vi "GPIB_SR400_B.vi"(11 "N per point":i32=1) -> (0 "B Gate":dbl[](array[numeric]), 2 "x/y":dbl)   [LabVIEW 2024]
uses:
  <vilib>/Utility/error.llb/Trim Whitespace One-Sided.vi
  GPIB_Address.vi
panel:
  in  "VISA resource name":refnum<visa-resource-name>="GPIB0::23::INSTR"
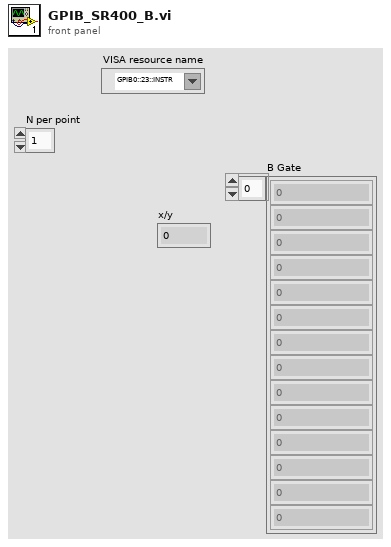
[diagram p1: front panel]
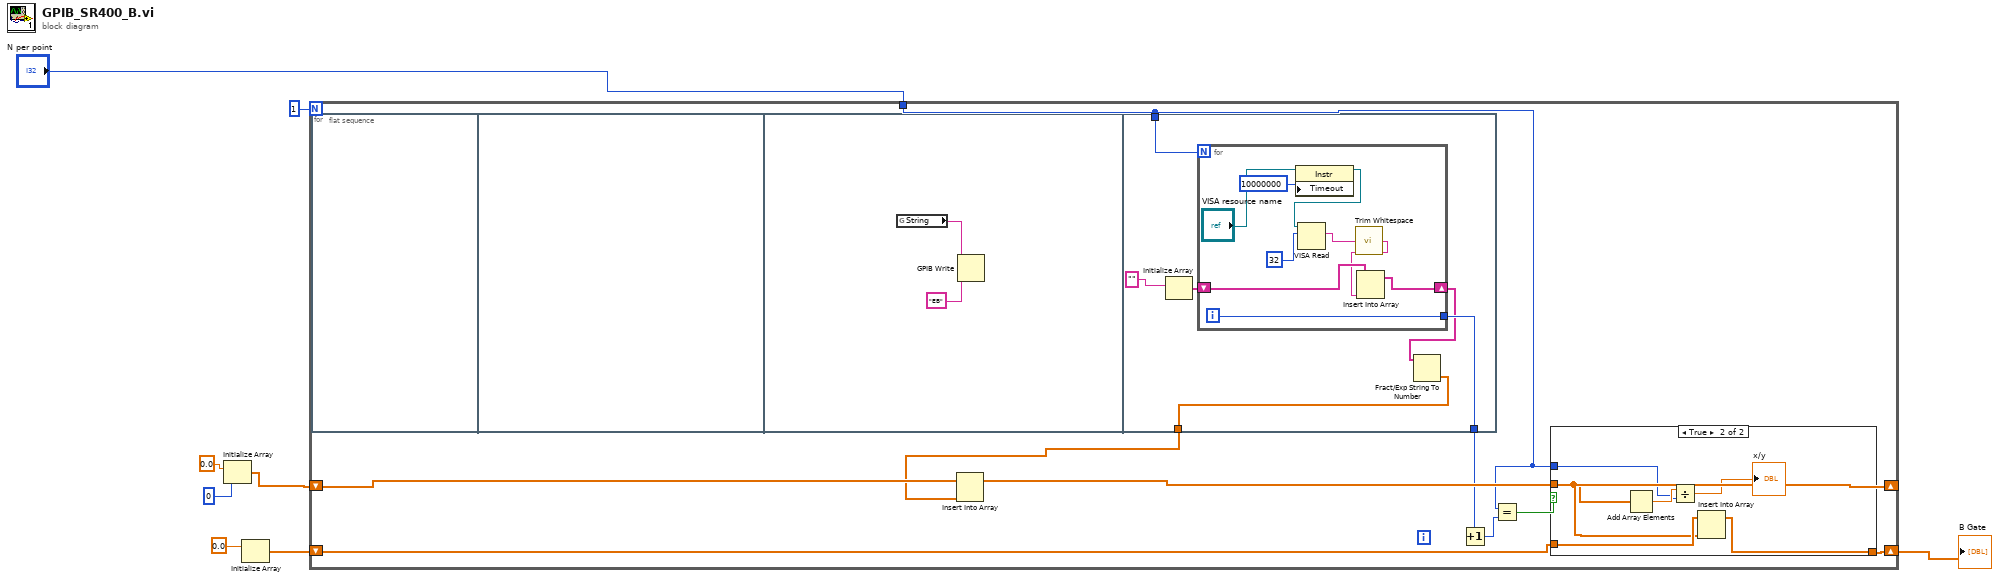
[diagram p0: block diagram]
diagram:
  n1 = Initialize Array(0.0, 0 ("dimension size")) -> (w8:dbl[])
  n2 = Initialize Array(0.0) -> (w6:dbl[])  [unwired: 1 in]
  n3 = for {
    N: 1 -> [_]
    shift-right: [w15] -> _
    shift-left: w8 -> [w17]
    shift-right: [w13] -> w5
    shift-left: w6 -> [w12]
    tunnel: "N per point" -> [w11]
    n4 = flat-sequence {
      tunnel: w11 -> [w31]
      tunnel: [w28] -> w10
      tunnel: [w26] -> w9
      frame #0 {
      }
      frame #1 {
      }
      frame #2 {
        n5 = global read "GPIB_Address.vi" "String"() -> (w24:string)
        n6 = GPIB Write(0:w24, 1:"EB" ("data")) -> ()  [unwired: 3 in, 2 out]
      }
      frame #3 {
        n7 = Initialize Array("") -> (w29:string[])  [unwired: 1 in]
        n8 = for {
          N: w31 -> [_]
          shift-right: [w38] -> w27
          shift-left: w29 -> [w39]
          tunnel: [w32] -> w28
          i -> [w32]
          n9 = property class="Instr"(reference="VISA resource name", "Timeout"=u32 10000000 ("General Settings:Timeout Value")) -> (reference out=w33:refnum<visa-resource-name>)  [unwired: 1 in, 1 out]
          n10 = VISA Read(VISA resource name=w33, byte count=32) -> (read buffer=w36:string)  [unwired: 1 in, 3 out]
          n11 = call <vilib>:"Trim Whitespace.vi"("string"=w36) -> ("trimmed string"=w37:string)  [unwired: 1 in]
          n12 = Insert Into Array "Insert Into Array"(array=w39, new element=w37) -> (w38:string[])  [unwired: 1 in]
        }
        n13 = Fract/Exp String To Number(string=w27) -> (number=w26:dbl[])  [unwired: 3 in, 1 out]
      }
    }
    n14 = Insert Into Array "Insert Into Array"(array=w17, new element=w9) -> (w15:dbl[])  [unwired: 1 in]
    n15 = Increment(x=w10) -> (x+1=w14:i32)
    n16 = Equal?(x=w11, y=w14) -> (x = y?=w16:bool)
    n17 = case shown="True" w16 {
      tunnel: w15 -> [_ w18]
      tunnel: w11 -> [_ w22]
      tunnel: [_ w19] -> w13
      tunnel: w12 -> [_ w20]
      frame False {
      }
      frame True {
        n18 = Add Array Elements(numeric array=w18) -> (sum=w23:dbl)
        n19 = Divide(x=w23, y=w22) -> (x/y=→"x/y":dbl)
        n20 = Insert Into Array(array=w20, new element=w18) -> (w19:dbl[])  [unwired: 1 in]
      }
    }
  }
  "B Gate" <- w5
